vi "UnscentedKalmanFilter_New.vi"(4 "Inputs":i32, 5 "States":i32, 6 "dt_Seconds":dbl=0.02, 7 "Outputs":i32, 8 "UNSCENTED_KALMAN_NEW_FUNC_GROUP":T1, 10 "MeasurementStdDevs":T3, 11 "StateStdDevs":T3) -> (0 "Error":errorcluster, 3 "UnscentedKalmanFiilter":T4)   [LabVIEW 2019, in "Trajectory_Library.lvlib"]
doc: "A Kalman filter combines predictions from a model and measurements to give an estimate of the true ystem state. This is useful because many states cannot be measured directly as a result of sensor noise, or because the state is \"hidden\".\n \nThe Unscented Kalman filter is similar to the Kalman filter, except that it propagates carefully chosen points called sigma points through the non-linear model to obtain an estimate of the true covariance (as opposed to a linearized version of it). This means that the UKF works with nonlinear systems.\n \nConstructs an unscented Kalman filter with custom mean, residual, and addition functions. Using custom functions for arithmetic can be useful if you have angles in the state or measurements, because they allow you to correctly account for the modular nature of angle arithmetic.\n \nInputs:\n - states -- The number of states.\n - outputs -- The number of outputs.\n - sstateStdDevs -- Standard deviations of model states.\n - measurementStdDevs -- Standard deviations of measurements.\n - nominalDtSeconds Nominal discretization timestep.\n - Inputs -- The number of inputs.\n - FunctionGroup -- A packed cluster containing the callback functions.\n\nOutputs:\n - outUnscentedKalmanFilter -- updated filter data cluster\n - Error -- If TRUE, and error occured."
uses:
  Trajectory_Library.lvlib
  <vilib>/Analysis/Matrix/Datatypes/RealMatrix.ctl
  <vilib>/Analysis/Matrix/NI_Matrix.lvlib
  TypeDef/MERWE_SCALED_SIGMA_PTS.ctl
  TypeDef/UNSCENTED_KALMAN_FILTER.ctl
  TypeDef/CALLBACK_FUNC_TYPE.ctl
  TypeDef/UNSCENTED_KALMAN_NEW_FUNC_GROUP.ctl
panel:
  # "<States,1>"
  # "<Outputs,1>"
  # "State Estimate <Statess,1>"
  # "<States, States>"
  # "<States, ?>"
  # "<Statess,  States>"
  # "<Outputs, Outputs>"
  # "<?, 1>"
  # "<?, 1>"
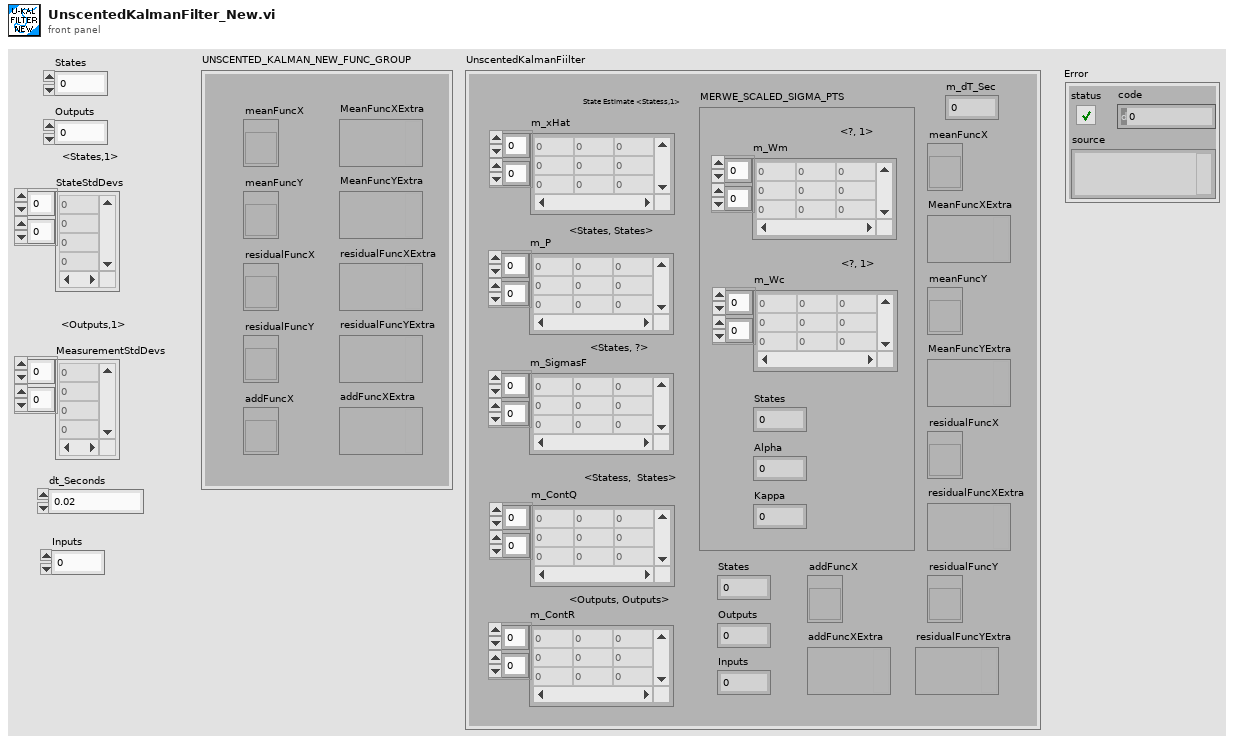
[diagram p1: front panel]
types:
  T1 = typedef "Trajectory_Library.lvlib/UNSCENTED_KALMAN_NEW_FUNC_GROUP.ctl" = cluster{"meanFuncX":T2, "meanFuncY":T2, "residualFuncX":T2, "residualFuncY":T2, "addFuncX":T2, "MeanFuncXExtra":variant, "MeanFuncYExtra":variant, "residualFuncXExtra":variant, "residualFuncYExtra":variant, "addFuncXExtra":variant}
  T2 = typedef "Trajectory_Library.lvlib/CALLBACK_FUNC_TYPE.ctl" = refnum<vi>
  T3 = typedef "NI_Matrix.lvlib/RealMatrix.ctl" = dbl[][]
  T4 = typedef "Trajectory_Library.lvlib/UNSCENTED_KALMAN_FILTER.ctl" = cluster{"m_P":T3, "m_xHat":T3, "States":i32, "Outputs":i32, "m_ContR":T3, "m_ContQ":T3, "m_SigmasF":T3, "m_dT_Sec":dbl, "MERWE_SCALED_SIGMA_PTS":T5, "meanFuncX":T2, "meanFuncY":T2, "residualFuncX":T2, "residualFuncY":T2, "addFuncX":T2, "addFuncXExtra":variant, "residualFuncYExtra":variant, "residualFuncXExtra":variant, "MeanFuncYExtra":variant, "MeanFuncXExtra":variant, "Inputs":i32}
  T5 = typedef "Trajectory_Library.lvlib/MERWE_SCALED_SIGMA_PTS.ctl" = cluster{"m_Wm":T3, "States":i32, "Alpha":dbl, "m_Wc":T3, "Kappa":i32}
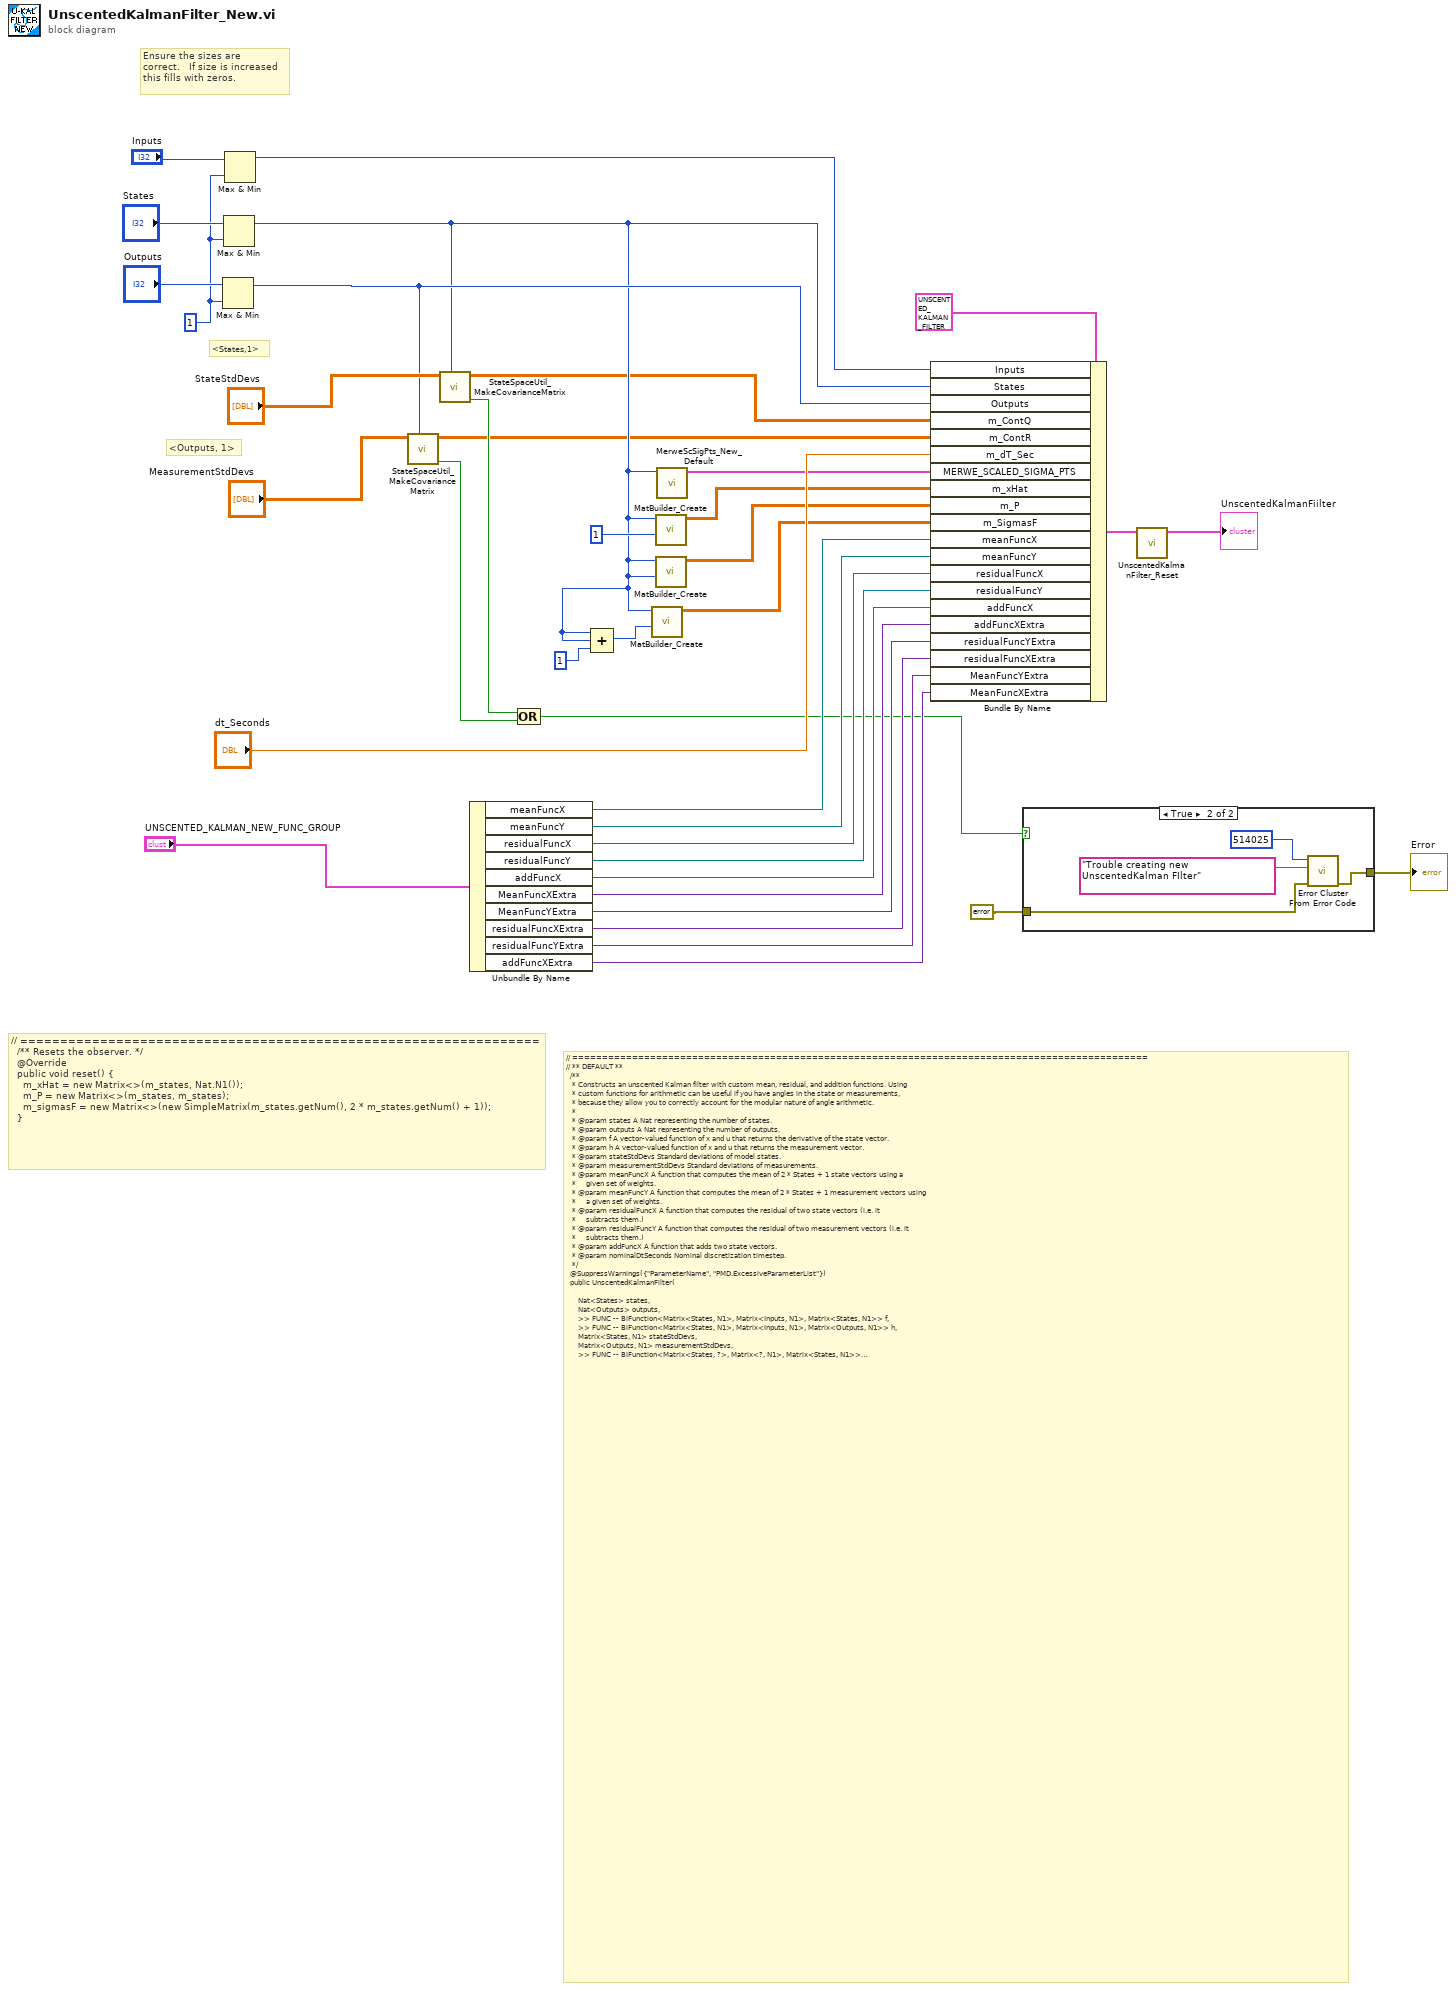
[diagram p0: block diagram]
diagram:
  w9 = 1 ("y")
  # "// =================================================================\n  /** Resets the observer. */\n  @Override\n  public void reset() {\n    m_xHat = new Matrix<>(m_states, Nat.N1());\n    m_P = new Matrix<>(m_states, m_states);\n    m_sigmasF = new Matrix<>(new SimpleMatrix(m_states.getNum(), 2 * m_states.getNum() + 1));\n  }"
  # "// ================================================================================================\n// ** DEFAULT **\n  /**\n   * Constructs an unscented Kalman filter with custom mean, residual, and addition functions. Using\n   * custom functions for arithmetic can be useful if you have angles in the state or measurements,\n   * because they allow you to correctly account for the modular nature of angle arithmetic.\n   *\n   * @param states A Nat representing the number of states.\n   * @param outputs A Nat representing the number of outputs.\n   * @param f A vector-valued function of x and u that returns the derivative of the state vector.\n   * @param h A vector-valued function of x and u that returns the measurement vector.\n   * @param stateStdDevs Standard deviations of model states.\n   * @param measurementStdDevs Standard deviations of measurements.\n   * @param meanFuncX A function that computes the mean of 2 * States + 1 state vectors using a\n   *     given set of weights.\n   * @param meanFuncY A function that computes the mean of 2 * States + 1 measurement vectors using\n   *     a given set of weights.\n   * @param residualFuncX A function that computes the residual of two state vectors (i.e. it\n   *     subtracts them.)\n   * @param residualFuncY A function that computes the residual of two measurement vectors (i.e. it\n   *     subtracts them.)\n   * @param addFuncX A function that adds two state vectors.\n   * @param nominalDtSeconds Nominal discretization timestep.\n   */\n  @SuppressWarnings({\"ParameterName\", \"PMD.ExcessiveParameterList\"})\n  public UnscentedKalmanFilter(\n\n      Nat<States> states,\n      Nat<Outputs> outputs,\n      >> FUNC -- BiFunction<Matrix<States, N1>, Matrix<Inputs, N1>, Matrix<States, N1>> f,\n      >> FUNC -- BiFunction<Matrix<States, N1>, Matrix<Inputs, N1>, Matrix<Outputs, N1>> h,\n      Matrix<States, N1> stateStdDevs,\n      Matrix<Outputs, N1> measurementStdDevs,\n      >> FUNC -- BiFunction<Matrix<States, ?>, Matrix<?, N1>, Matrix<States, N1>> meanFuncX,\n      >> FUNC -- BiFunction<Matrix<Outputs, ?>, Matrix<?, N1>, Matrix<Outputs, N1>> meanFuncY,\n      >> FUNC -- BiFunction<Matrix<States, N1>, Matrix<States, N1>, Matrix<States, N1>> residualFuncX,\n      >> FUNC -- BiFunction<Matrix<Outputs, N1>, Matrix<Outputs, N1>, Matrix<Outputs, N1>> residualFuncY,\n      >> FUNC -- BiFunction<Matrix<States, N1>, Matrix<States, N1>, Matrix<States, N1>> addFuncX,\n      double nominalDtSeconds) {\n\n    this.m_states = states;\n    this.m_outputs = outputs;\n\n    m_f = f;\n    m_h = h;\n\n    m_meanFuncX = meanFuncX;\n    m_meanFuncY = meanFuncY;\n    m_residualFuncX = residualFuncX;\n    m_residualFuncY = residualFuncY;\n    m_addFuncX = addFuncX;\n\n    m_dtSeconds = nominalDtSeconds;\n\n    m_contQ = StateSpaceUtil.makeCovarianceMatrix(states, stateStdDevs);\n    m_contR = StateSpaceUtil.makeCovarianceMatrix(outputs, measurementStdDevs);\n\n    m_pts = new MerweScaledSigmaPoints<>(states);\n\n    reset();\n  }"
  # "<Outputs, 1>"
  # "<States,1>"
  # "Ensure the sizes are\ncorrect.   If size is increased \nthis fills with zeros."
  n1 = Max & Min(x="Outputs", y=w9) -> (max(x,y)=w32:i32)  [unwired: 1 out]
  n2 = Max & Min(x="States", y=w9) -> (max(x,y)=w24:i32)  [unwired: 1 out]
  n3 = Max & Min(x="Inputs", y=w9) -> (max(x,y)=w8:i32)  [unwired: 1 out]
  n4 = call "StateSpaceUtil_MakeCovarianceMatrix.vi"("States"=w32, "StdDevs"="MeasurementStdDevs") -> ("Size Coerced"=w6:bool, "Covariance Matrix"=w4:T3)  [unwired: 8 in]
  n5 = call "StateSpaceUtil_MakeCovarianceMatrix.vi"("States"=w24, "StdDevs"="StateStdDevs") -> ("Size Coerced"=w7:bool, "Covariance Matrix"=w5:T3)  [unwired: 8 in]
  n6 = Unbundle By Name("UNSCENTED_KALMAN_NEW_FUNC_GROUP") -> ("meanFuncX"=w20:T2, "meanFuncY"=w19:T2, "residualFuncX"=w18:T2, "residualFuncY"=w17:T2, "addFuncX"=w16:T2, "MeanFuncXExtra"=w15:variant, "MeanFuncYExtra"=w14:variant, "residualFuncXExtra"=w13:variant, "residualFuncYExtra"=w12:variant, "addFuncXExtra"=w11:variant)
  n7 = Compound Arithmetic op=OR(w7, w6) -> (w3:bool)
  n8 = Compound Arithmetic op=ADD(w24, w24, 1 ("value")) -> (w23:i32)
  n9 = call "MatBuilder_Create.vi"("Columns"=w23, "Rows"=w24) -> ("output matrix"=w22:T3)  [unwired: 9 in]
  n10 = call "MatBuilder_Create.vi"("Columns"=1, "Rows"=w24) -> ("output matrix"=w27:T3)  [unwired: 9 in]
  n11 = call "MatBuilder_Create.vi"("Columns"=w24, "Rows"=w24) -> ("output matrix"=w26:T3)  [unwired: 9 in]
  n12 = call "MerweScSigPts_New_Default.vi"("States"=w24) -> ("MerweScaledSigmaPts"=w31:T5)  [unwired: 10 in]
  n13 = Bundle By Name(cluster=T4 {"m_P"=[], "m_xHat"=[], "States"=0, "Outputs"=0, "m_ContR"=[], "m_ContQ"=[], "m_SigmasF"=[], "m_dT_Sec"=0.0, "MERWE_SCALED_SIGMA_PTS"={"m_Wm"=[], "States"=0, "Alpha"=0.0, "m_Wc"=[], "Kappa"=0}, "meanFuncX"=refnum, "meanFuncY"=refnum, "residualFuncX"=refnum, "residualFuncY"=refnum, "addFuncX"=refnum, "addFuncXExtra"=variant, "residualFuncYExtra"=variant, "residualFuncXExtra"=variant, "MeanFuncYExtra"=variant, "MeanFuncXExtra"=variant, "Inputs"=0} ("UNSCENTED_KALMAN_FILTER"), "Inputs"=w8, "States"=w24, "Outputs"=w32, "m_ContQ"=w5, "m_ContR"=w4, "m_dT_Sec"="dt_Seconds", "MERWE_SCALED_SIGMA_PTS"=w31, "m_xHat"=w27, "m_P"=w26, "m_SigmasF"=w22, "meanFuncX"=w20, "meanFuncY"=w19, "residualFuncX"=w18, "residualFuncY"=w17, "addFuncX"=w16, "addFuncXExtra"=w15, "residualFuncYExtra"=w14, "residualFuncXExtra"=w13, "MeanFuncYExtra"=w12, "MeanFuncXExtra"=w11) -> (w30:T4)
  n14 = case shown="True" w3 {
    tunnel: errorcluster {"status"=FALSE, "code"=0, "source"=""} ("error constant") -> [w39 w42]
    tunnel: [w39 w43] -> w1
    frame False {
    }
    frame True {
      n15 = call <vilib>:"Error Cluster From Error Code.vi"("error in (no error)"=w42, "error message (\"\")"="Trouble creating new UnscentedKalman FIlter" ("error message (\"\")"), "error code (0)"=514025) -> ("error out"=w43:errorcluster)  [unwired: 6 in]
    }
  }
  "Error" <- w1
  n16 = call "UnscentedKalmanFilter_Reset.vi"("in UnscentedKalmanFiilter"=w30) -> ("out UnscentedKalmanFiilter"=→"UnscentedKalmanFiilter":T4)  [unwired: 10 in]
